vi "UnscentedKalmanFilter_GetXHat_Single.vi"(10 "Row":i32, 11 "in UnscentedKalmanFiilter":T1) -> (3 "xHat Value":dbl)   [LabVIEW 2019, in "Trajectory_Library.lvlib"]
doc: "Returns an element of the state estimate x-hat.\n \nInputs:\n - inUnscentedKalmanFilter -- filter data cluster\n - row -- Row of x-hat.\n\nOutputs:\n - xHat_Value -- the value of the state estimate x-hat at i."
uses:
  Trajectory_Library.lvlib
  <vilib>/Analysis/Matrix/Datatypes/RealMatrix.ctl
  <vilib>/Analysis/Matrix/NI_Matrix.lvlib
  TypeDef/MERWE_SCALED_SIGMA_PTS.ctl
  TypeDef/UNSCENTED_KALMAN_FILTER.ctl
  TypeDef/CALLBACK_FUNC_TYPE.ctl
panel:
  # "State Estimate <Statess,1>"
  # "<States, States>"
  # "<States, ?>"
  # "<Statess,  States>"
  # "<Outputs, Outputs>"
  # "<?, 1>"
  # "<?, 1>"
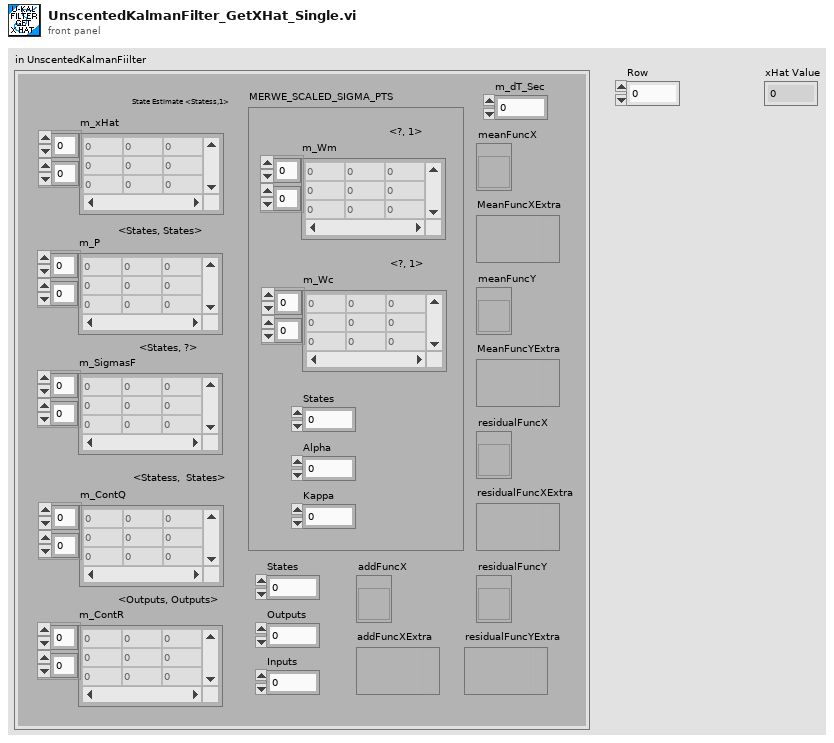
[diagram p1: front panel]
types:
  T1 = typedef "Trajectory_Library.lvlib/UNSCENTED_KALMAN_FILTER.ctl" = cluster{"m_P":T2, "m_xHat":T2, "States":i32, "Outputs":i32, "m_ContR":T2, "m_ContQ":T2, "m_SigmasF":T2, "m_dT_Sec":dbl, "MERWE_SCALED_SIGMA_PTS":T3, "meanFuncX":T4, "meanFuncY":T4, "residualFuncX":T4, "residualFuncY":T4, "addFuncX":T4, "addFuncXExtra":variant, "residualFuncYExtra":variant, "residualFuncXExtra":variant, "MeanFuncYExtra":variant, "MeanFuncXExtra":variant, "Inputs":i32}
  T2 = typedef "NI_Matrix.lvlib/RealMatrix.ctl" = dbl[][]
  T3 = typedef "Trajectory_Library.lvlib/MERWE_SCALED_SIGMA_PTS.ctl" = cluster{"m_Wm":T2, "States":i32, "Alpha":dbl, "m_Wc":T2, "Kappa":i32}
  T4 = typedef "Trajectory_Library.lvlib/CALLBACK_FUNC_TYPE.ctl" = refnum<vi>
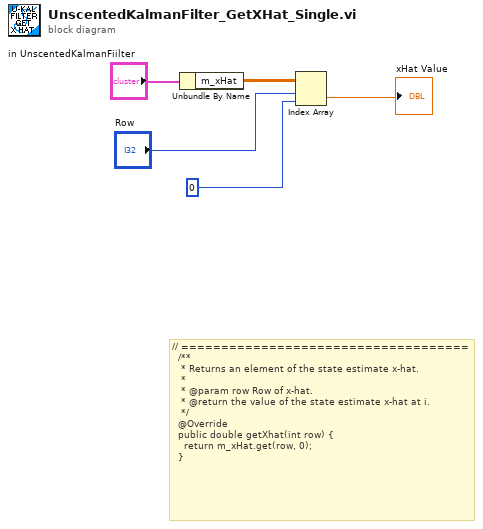
[diagram p0: block diagram]
diagram:
  # "// ====================================\n  /**\n   * Returns an element of the state estimate x-hat.\n   *\n   * @param row Row of x-hat.\n   * @return the value of the state estimate x-hat at i.\n   */\n  @Override\n  public double getXhat(int row) {\n    return m_xHat.get(row, 0);\n  }"
  n1 = Unbundle By Name("in UnscentedKalmanFiilter") -> ("m_xHat"=w5:T2)
  n2 = Index Array(array=w5, index (row)="Row", index (col)=0) -> (element=→"xHat Value":dbl)
